vi "test_Basic Waveform Read.vi"(8 "error in (no error)":errorcluster, 11 "DMA Channels Basic Testing in":refnum<class "FPGA Addon DMA Channels Interleaved System Tests.lvclass">) -> (0 "error out":errorcluster, 3 "DMA Channels Basic Testing out":refnum<class "FPGA Addon DMA Channels Interleaved System Tests.lvclass">)   [LabVIEW 2020, in "FPGA Addon DMA Channels Interleaved System Tests.lvclass"]
uses:
  FPGA Addon DMA Channels Interleaved System Tests.lvclass
  FPGA Addon Test Class/FPGA Addon Test Class.lvclass
panel:
  out "Waveform":waveform(dbl)(graph)
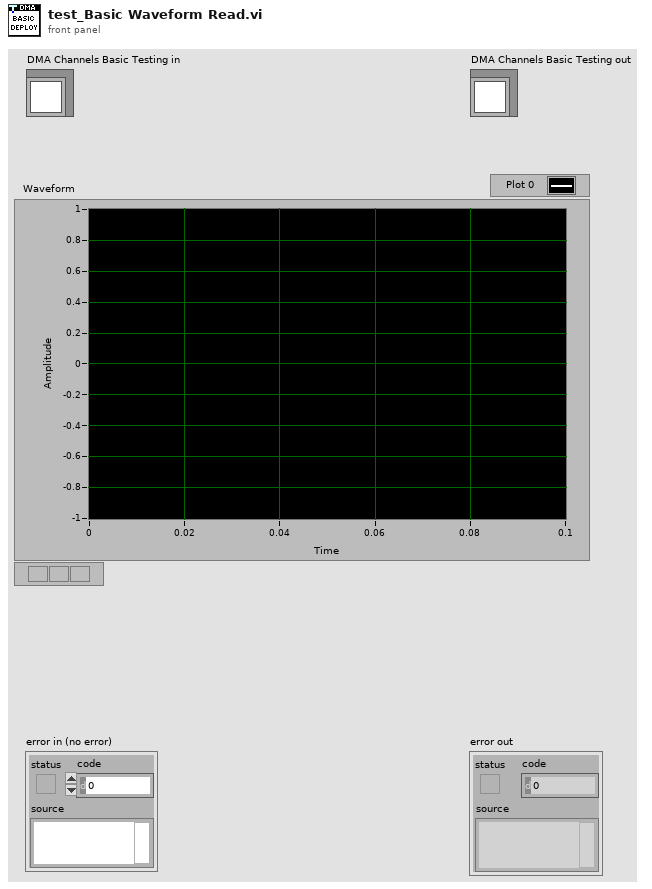
[diagram p1: front panel]
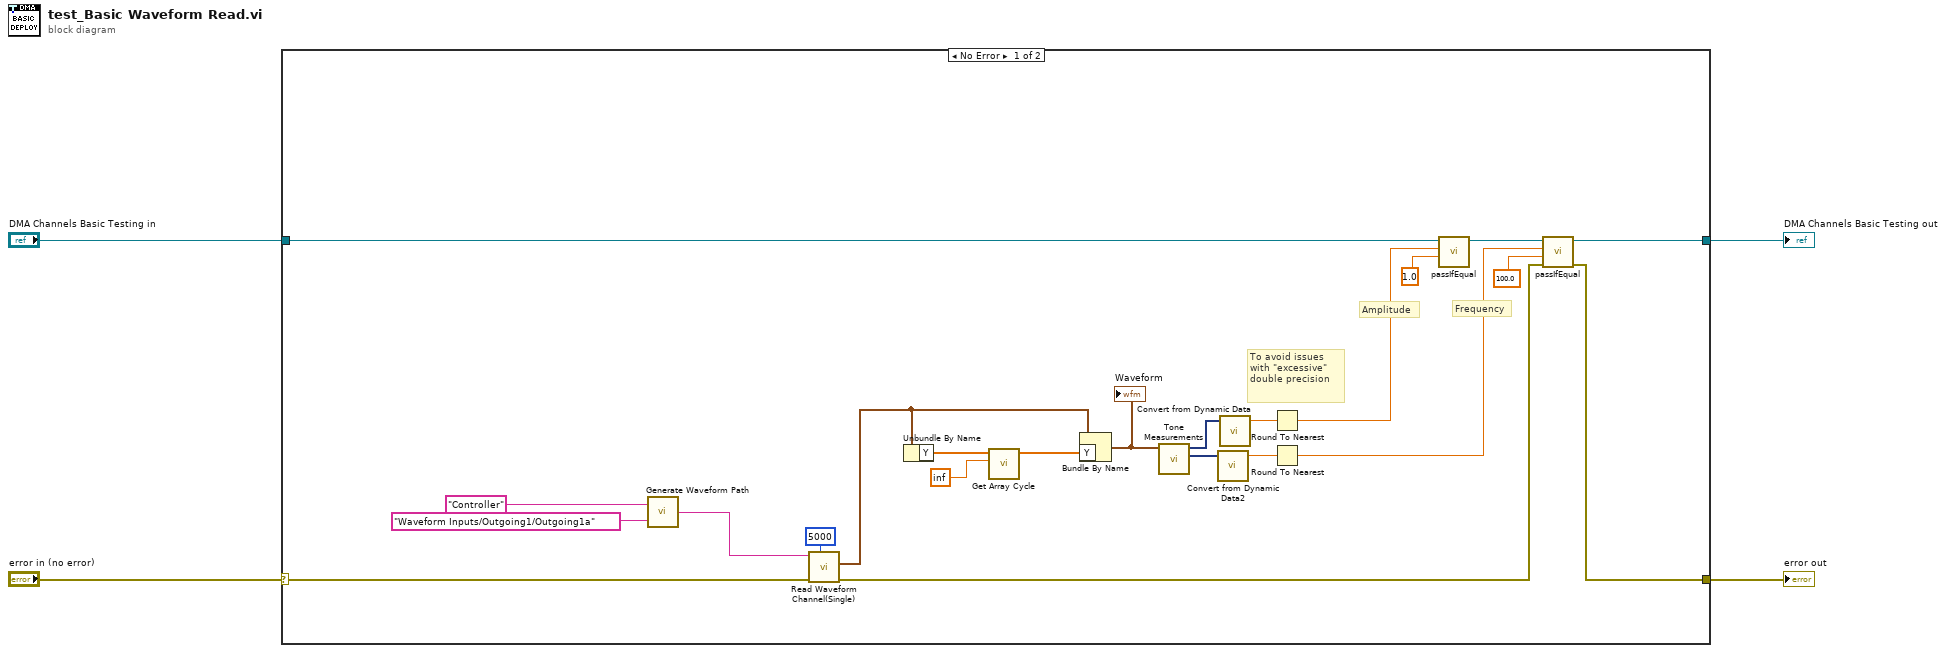
[diagram p0: block diagram]
diagram:
  n1 = case shown="No Error" "error in (no error)" {
    selector: "error in (no error)" -> [w26 w28]
    tunnel: "DMA Channels Basic Testing in" -> [w11 w29]
    tunnel: [w25 w29] -> w3
    tunnel: [w23 w28] -> w2
    frame No Error {
      # "To avoid issues with \"excessive\" double precision"
      # "Frequency"
      # "Amplitude"
      n2 = call "Generate Waveform Path.vi"("Relative Waveform Path"="Waveform Inputs/Outgoing1/Outgoing1a", "Target Name"="Controller") -> ("Waveform Path Out"=w5:string)
      n3 = call "Read Waveform Channel(Single).vi"("Timeout"=5000, "error in (no error)"=w26, "Waveform path in"=w5) -> ("error out"=w24:errorcluster, "Waveform data"=w20:waveform(dbl))  [unwired: 6 in, 1 out]
      n4 = Unbundle By Name(w20) -> ("Y"=w22:dbl[])
      n5 = call "Get Array Cycle.vi"("Marker"=inf, "Array Samples"=w22) -> ("Array"=w19:dbl[])  [unwired: 8 in, 1 out]
      n6 = Bundle By Name(cluster=w20, "Y"=w19) -> (w18:waveform(dbl))
      "Waveform" <- w18
      n7 = call "Tone Measurements"("Signals"=w18) -> ("Frequency"=w17:dynamicdata, "Amplitude"=w15:dynamicdata)  [unwired: 8 in, 1 out]
      n8 = call "Convert from Dynamic Data2"("Dynamic Data Type"=w17) -> ("Scalar"=w13:dbl)  [unwired: 3 in]
      n9 = call "Convert from Dynamic Data"("Dynamic Data Type"=w15) -> ("Scalar"=w14:dbl)  [unwired: 3 in]
      n10 = Round To Nearest(number=w14) -> (nearest integer value=w10:dbl)
      n11 = Round To Nearest(number=w13) -> (nearest integer value=w12:dbl)
      n12 = call-dynamic "passIfEqual.vi"("y"=1.0 ("Scalar"), "x"=w10, "TestCase in"=w11) -> ("TestCase out"=w8:refnum<class "FPGA Addon DMA Channels Interleaved System Tests.lvclass">)  [unwired: 7 in, 1 out]
      n13 = call-dynamic "passIfEqual.vi"("error in (no error)"=w24, "y"=100.0 ("Scalar"), "x"=w12, "TestCase in"=w8) -> ("error out"=w23:errorcluster, "TestCase out"=w25:refnum<class "FPGA Addon DMA Channels Interleaved System Tests.lvclass">)  [unwired: 6 in]
    }
    frame Error {
    }
  }
  "error out" <- w2
  "DMA Channels Basic Testing out" <- w3
